vi "Initialize from Teststand.vi"(4 "error in (no error)":errorcluster, 7 "Engine Reference":refnum<k7>) -> (0 "error out":errorcluster, 3 "EasyUserManager out":refnum<class "EasyUserManager.lvclass">)   [LabVIEW 2024, in "EasyUserManager.lvclass"]
doc: "Create a new <B>EasyUserManager</B> object instance and set the provided Teststand Engine to the class attribute.\n\nThe provided Engine reference is duplicated to avoid automatic closing of the reference when the VI completes executing. Use this VI to initialize an EasyUserManager object from Teststand."
uses:
  EasyUserManager.lvclass
  EasyUserManager.lvclass/EasyUserManager.ctl
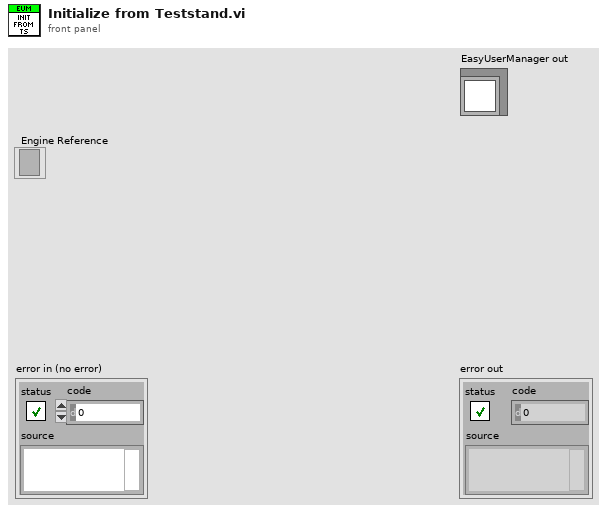
[diagram p1: front panel]
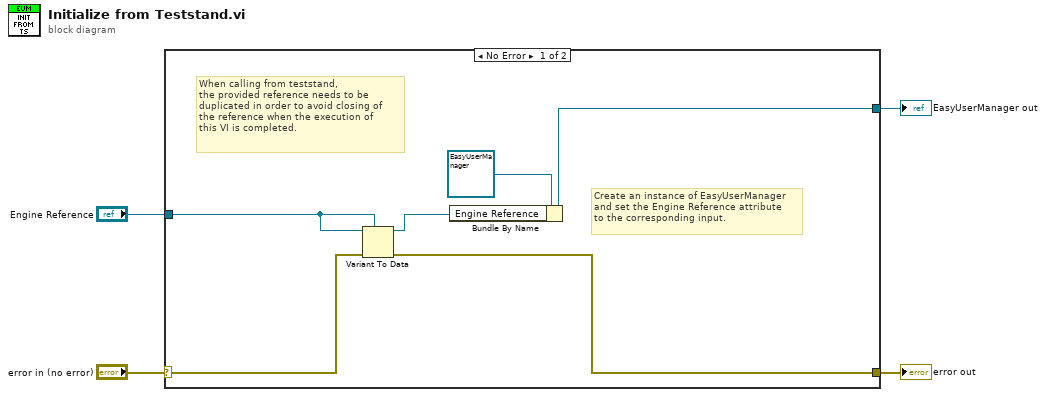
[diagram p0: block diagram]
diagram:
  n1 = case shown="No Error" "error in (no error)" {
    selector: "error in (no error)" -> [w6 w11]
    tunnel: [w5 w11] -> w3
    tunnel: [w10 _] -> w2
    tunnel: "Engine Reference" -> [w8 _]
    frame No Error {
      # "When calling from teststand,\nthe provided reference needs to be\nduplicated in order to avoid closing of \nthe reference when the execution of\nthis VI is completed."
      # "Create an instance of EasyUserManager\nand set the Engine Reference attribute\nto the corresponding input."
      n2 = Variant To Data(error in=w6, type=w8, Variant=w8) -> (data=w7:refnum<k7>, error out=w5:errorcluster)
      n3 = Bundle By Name(cluster=refnum<class "EasyUserManager.lvclass"> refnum ("EasyUserManager.lvclass"), "Engine Reference"=w7) -> (w10:refnum<class "EasyUserManager.lvclass">)
    }
    frame Error {
      # "Pass error and do nothing."
    }
  }
  "error out" <- w3
  "EasyUserManager out" <- w2
